vi "Cancel Requested.vi"(8 "error in":errorcluster) -> (0 "error out":errorcluster, 3 "cancelled?":bool)   [LabVIEW 2020, in "MCP Server.lvlib"]
doc: "Call this from a tool VI that works in a loop without reporting progress, to learn whether the client has given up. cancelled? TRUE: stop and return; the server sends nothing more for this request.\n\n- Streamed tools/call (the client sent params._meta.progressToken and accepts text/event-stream): at most every 500 ms this sends an SSE comment \":\" (a keep-alive the client ignores) and waits up to 1 s for the stream to take it; when it does not, the client closed the stream, which is how a client cancels over HTTP in MCP 2026-07-28. Between those probes it returns the last known state at once, so it is cheap to call in a tight loop.\n- Legacy (MCP 2025-06-18 and older): also TRUE when the client sent notifications/cancelled with the id of this request. That arrives at once while the call is streamed; for a call that is not streamed it cannot arrive while the call runs (Process HTTP Request.vi handles one request at a time), so it has no effect.\n- Otherwise FALSE.\n\ncancelled? stays TRUE for the rest of the request."
uses:
  MCP Server.lvlib
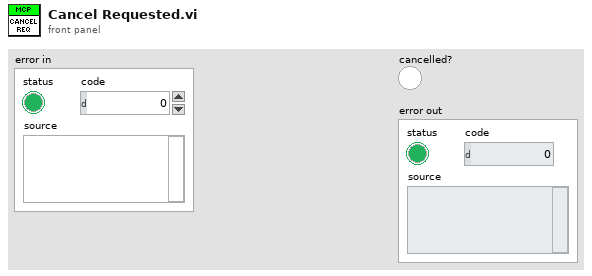
[diagram p1: front panel]
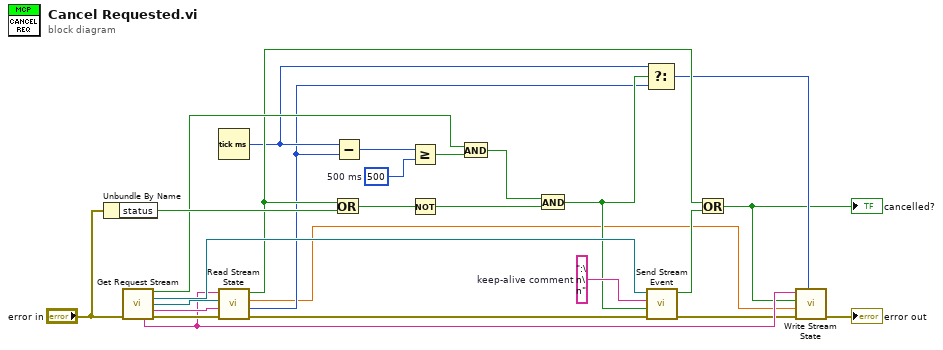
[diagram p0: block diagram]
diagram:
  w22 = u32 500  # 500 ms
  w13 = ":\n\n"  # keep-alive comment
  n1 = Unbundle By Name("error in") -> ("status"=w20:bool)
  n2 = call "Get Request Stream.vi"("error in"="error in") -> ("streaming?"=w18:bool, "events"=w14:refnum<queue>, "cancelled"=w26:refnum<queue>, "request id"=w25:string, "stream key"=w6:string, "error out"=w24:errorcluster)  [unwired: 8 in, 1 out]
  n3 = Tick Count (ms)() -> (millisecond timer value=w9:u32)
  n4 = call "Read Stream State.vi"("error in"=w24, "request id"=w25, "cancelled"=w26, "stream key"=w6) -> ("error out"=w12:errorcluster, "last probe"=w7:u32, "last progress"=w5:dbl, "cancelled?"=w11:bool)  [unwired: 4 in]
  n5 = Or(x=w11, y=w20) -> (x .or. y?=w19:bool)
  n6 = Subtract(x=w9, y=w7) -> (x-y=w23:u32)
  n7 = Greater Or Equal?(x=w23, y=w22) -> (x >= y?=w17:bool)
  n8 = Not(x=w19) -> (.not. x?=w15:bool)
  n9 = And(x=w18, y=w17) -> (x .and. y?=w16:bool)
  n10 = And(x=w16, y=w15) -> (x .and. y?=w8:bool)
  n11 = Select(t=w9, s=w8, f=w7) -> (s? t:f=w4:u32)
  n12 = call "Send Stream Event.vi"("error in"=w12, "send?"=w8, "event"=w13, "events"=w14) -> ("error out"=w3:errorcluster, "client gone?"=w10:bool)  [unwired: 6 in]
  n13 = Or(x=w11, y=w10) -> (x .or. y?=w2:bool)
  "cancelled?" <- w2
  n14 = call "Write Stream State.vi"("last probe"=w4, "error in"=w3, "last progress"=w5, "cancelled?"=w2, "stream key"=w6) -> ("error out"=→"error out":errorcluster)  [unwired: 6 in]
